vi "Create array.vi"(8 "error in (no error)":errorcluster, 9 "Name":string, 10 "ArrayObject":refnum<class "json class.lvclass">[](array[class]), 11 "json class in":refnum<class "json class.lvclass">) -> (0 "error out":errorcluster, 3 "json class out":refnum<class "json class.lvclass">)   [LabVIEW 2021, in "Config Library.lvlib" / "json class.lvclass"]
uses:
  json class.lvclass
  <vilib>/addons/JSON API/JSON Value/JSON Value.lvclass
  json class.lvclass/json class.ctl
  <vilib>/addons/JSON API/JSON Object/Set Object Item by name.vi
  <vilib>/addons/JSON API/JSON Object/JSON Object.lvclass
  C:/Program Files (x86)/National Instruments/LabVIEW 2021/vi.lib/addons/JSON API/JSON Value/JSON Value.lvclass
  <vilib>/addons/JSON API/JSON Array/JSON Array.lvclass
  <vilib>/addons/JSON API/JSON Array/Set JSON Array.vi
  <vilib>/addons/JSON API/Get Polymorphic/JSON GetSet.lvlib
  C:/Program Files (x86)/National Instruments/LabVIEW 2021/vi.lib/addons/JSON API/JSON Array/JSON Array.lvclass
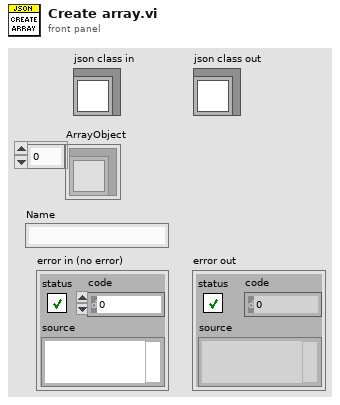
[diagram p1: front panel]
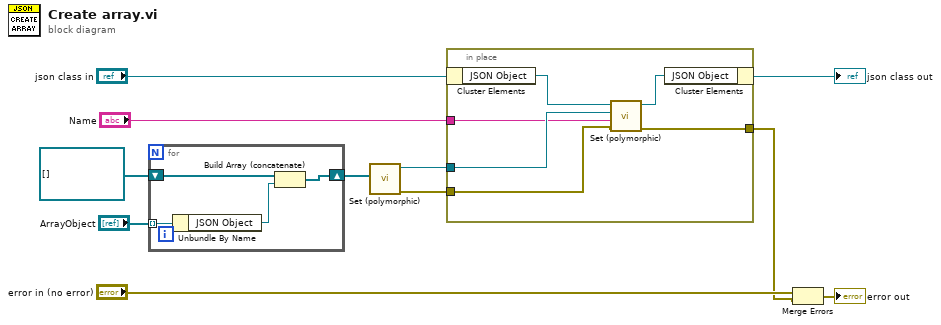
[diagram p0: block diagram]
diagram:
  n1 = for {
    tunnel: "ArrayObject" -> [w13] mode=indexing
    shift-right: [w15] -> w1
    shift-left: refnum<class "JSON Value.lvclass">[] [] ("Array") -> [w14]
    n2 = Unbundle By Name(w13) -> ("JSON Object"=w12:refnum<class "JSON Object.lvclass">)
    n3 = Build Array (concatenate)(w14, w12) -> (w15:refnum<class "JSON Value.lvclass">[])
  }
  n4 = call-poly <vilib>:"Set (polymorphic).vi"("Array"=w1) -> ("error out"=w5:errorcluster, "JSON Array out"=w7:refnum<class "JSON Array.lvclass">)  [unwired: 9 in]
  n5 = in-place {
    in-place-border: [w20] -> w6
    in-place-border: w7 -> [w19]
    in-place-border: w5 -> [w18]
    in-place-border: "Name" -> [w17]
    n6 = in-place-cluster #1("json class in") -> ("JSON Object"=w16:refnum<class "JSON Object.lvclass">)
    n7 = call-poly <vilib>:"Set (polymorphic).vi"("error in (no error)"=w18, "name"=w17, "Value"=w19, "JSON Object in"=w16) -> ("error out"=w20:errorcluster, "JSON Object out"=w21:refnum<class "JSON Object.lvclass">)  [unwired: 5 in, 1 out]
    n8 = in-place-cluster #1("JSON Object"=w21) -> (→"json class out":refnum<class "json class.lvclass">)
  }
  n9 = Merge Errors("error in (no error)", w6) -> (→"error out":errorcluster)
